vi "Initialise.vi"(8 "error in (no error)":errorcluster, 11 "Node in":refnum<class "bt_Parallel.lvclass">) -> (0 "error out":errorcluster, 3 "Node out":refnum<class "bt_Parallel.lvclass">)   [LabVIEW 2021, in "BT.lvlib" / "bt_Parallel.lvclass"]
uses:
  bt_Parallel.lvclass
  C:/Users/Tim/Documents/GitHub/LV_Behaviour_Tree/Source/Support/Nodes/Composites/abs_Composite/bt_Composite.lvclass
  abs_Node/Status.ctl
  abs_Composite/bt_Composite.lvclass/bt_Composite.ctl
  bt_Parallel.lvclass/bt_Parallel.ctl
  abs_Composite/Properties/Read Num Nodes.vi
  abs_Composite/bt_Composite.lvclass
  abs_Node/bt_Node.lvclass
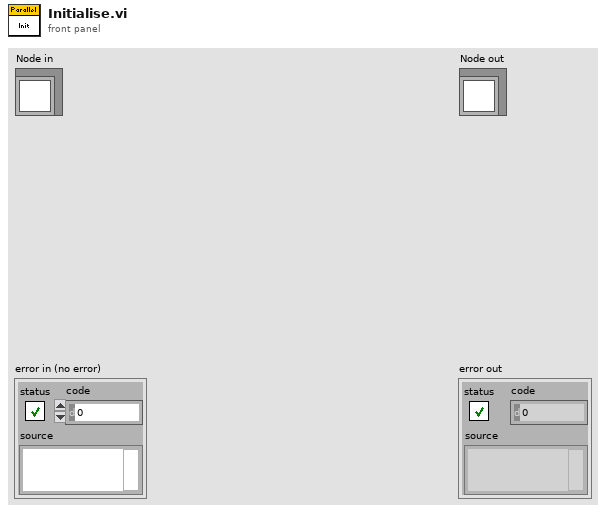
[diagram p1: front panel]
types:
  T1 = typedef "BT.lvlib/bt_Node.lvclass/Status.ctl" = enum16{"Success", "Failure", "Running"}
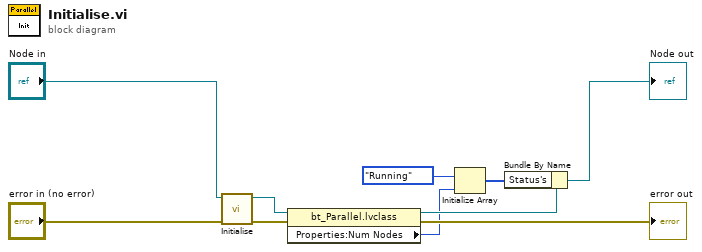
[diagram p0: block diagram]
diagram:
  n1 = call-parent "Initialise.vi"("error in (no error)"="error in (no error)", "Node in"="Node in") -> ("error out"=w6:errorcluster, "Node out"=w5:refnum<class "bt_Parallel.lvclass">)  [unwired: 8 in]
  n2 = property class="bt_Parallel.lvclass"(reference=w5, error in=w6) -> (reference out=w4:refnum<class "bt_Parallel.lvclass">, error out=→"error out":errorcluster, "Properties:Num Nodes"=w3:i32)
  n3 = Initialize Array(Status."Running" ("Status"), w3) -> (w1:T1[])
  n4 = Bundle By Name(cluster=w4, "Status's"=w1) -> (→"Node out":refnum<class "bt_Parallel.lvclass">)
